vi "Measure.vi"() -> ()   [LabVIEW 2024]
uses:
  <vilib>/MakerHub/LINX/Public/Peripherals/Analog/Analog Read N Chans.vi
  <vilib>/MakerHub/LINX/Public/Peripherals/PWM/PWM Set Duty Cycle 1 Chan.vi
  <vilib>/MakerHub/LINX/Private/Local IO/LinxAnalogRead.vi
  <vilib>/MakerHub/LINX/Public/Utilities/Check Channel.vi
  <vilib>/MakerHub/LINX/Public/Utilities/Open Serial.vi
  Globals.vi
  <vilib>/MakerHub/LINX/Public/Peripherals/PWM/PWM Set Duty Cycle N Chans.vi
  <vilib>/addons/control/pid/pid.llb/PID (DBL).vi
  <vilib>/MakerHub/LINX/Private/Utilties/Generate Error.vi
  <vilib>/Utility/file.llb/Write Delimited Spreadsheet (string).vi
  <vilib>/MakerHub/LINX/LMH-LINX.lvlib
  <vilib>/addons/control/pid/NI_PID_pid.lvlib
  <vilib>/Analysis/NI_AALBase.lvlib
panel:
  out "Resistance":dbl(graph)
  out "TREF 2 Error":dbl
  out "TREF 2":dbl
  out "TREF 1 Error":dbl
  out "SC":dbl
  out "TREF 1":dbl
  in  "Target TC":dbl format="%.2f"
  in  "Target TH":dbl format="%.2f"
  out "Auto":bool
  in  "Start Auto":bool
  in  "TH End":dbl(knob)=100.0 step=10.0 scale=0.0..100.0
  in  "TH Start":dbl(knob)=40.0 step=10.0 scale=0.0..100.0
  out "VOUT - 1.25":dbl(knob) scale=-1.0..1.0
  out "TC":dbl(slide) scale=0.0..100.0
  out "TH":dbl(slide) scale=0.0..100.0
  out "Voltage":dbl(graph)
  out "TH":dbl(graph)
  in  "Save to File":bool
  out "VOUT - 1.25":dbl
  out "TC":dbl(graph)
  out "TC":dbl
  in  "Stop Button":bool
  out "TH":dbl
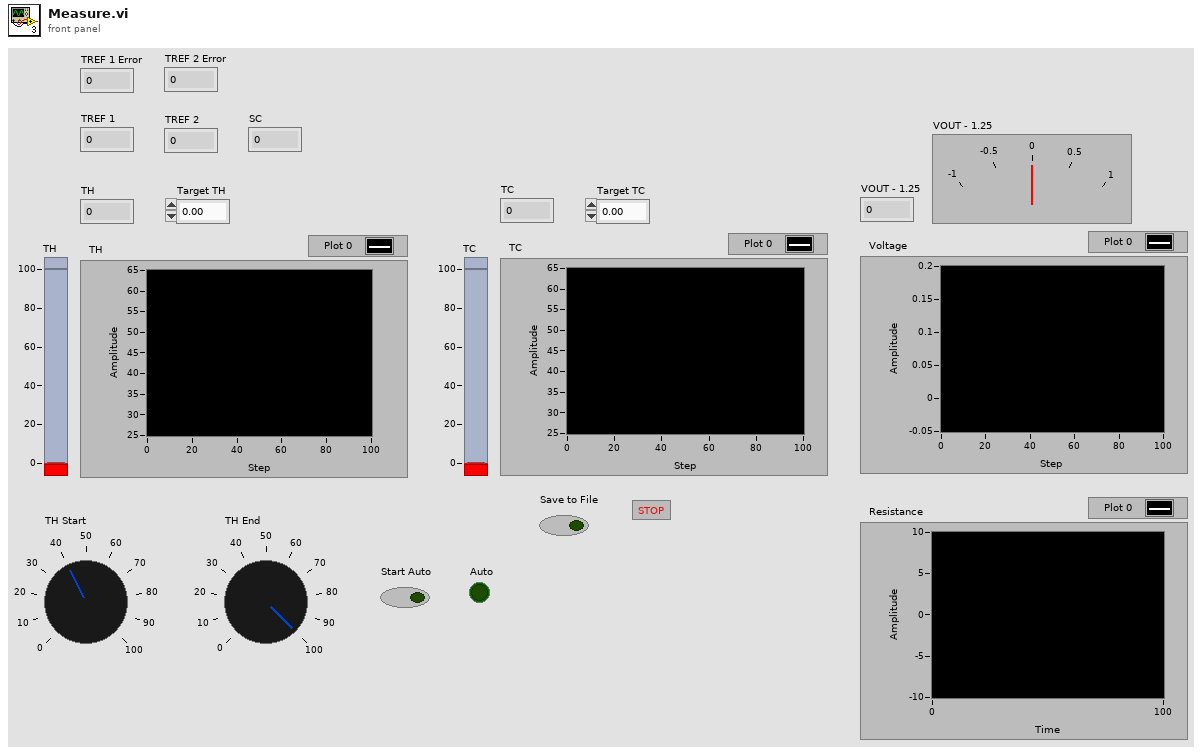
[diagram p1: front panel]
types:
  T1 = typedef "LMH-LINX.lvlib/LINX Ref.ctl" = cluster{"IO":T2, "Interface":T3, "LINX Device Config":T4}
  T2 = typedef "LMH-LINX.lvlib/Platform.ctl" = enum16{"Remote", "Local"}
  T3 = typedef "LMH-LINX.lvlib/Interface.ctl" = enum16{"Serial", "TCP"}
  T4 = typedef "LMH-LINX.lvlib/Device.lvlib/LINX Device Config.ctl" = cluster{"Interface":T3, "COM Port":refnum<visa-resource-name>, "TCP Configuration":T5, "Device Family":u8, "Device ID":u8, "Device Name":string, "TCP Ref":refnum<k5>, "Channels":T6}
  T5 = typedef "LMH-LINX.lvlib/Device.lvlib/TCP Config.ctl" = cluster{"IP Address":string, "Port":u16}
  T6 = typedef "LMH-LINX.lvlib/Channels.ctl" = cluster{"DI":u8[], "DO":u8[], "AI":u8[], "AO":u8[], "PWM":u8[], "QE":u8[], "UART":u8[], "I2C 2":u8[], "SPI":u8[], "CAN":u8[], "Servo":u8[], "AI Ref (V)":dbl, "AI Resolution (Bits)":u8, "AO Ref (V)":dbl, "AO Resolution (Bits)":u8}
  T7 = cluster{"proportional gain (Kc)":dbl, "integral time (Ti, min)":dbl, "derivative time (Td, min)":dbl}
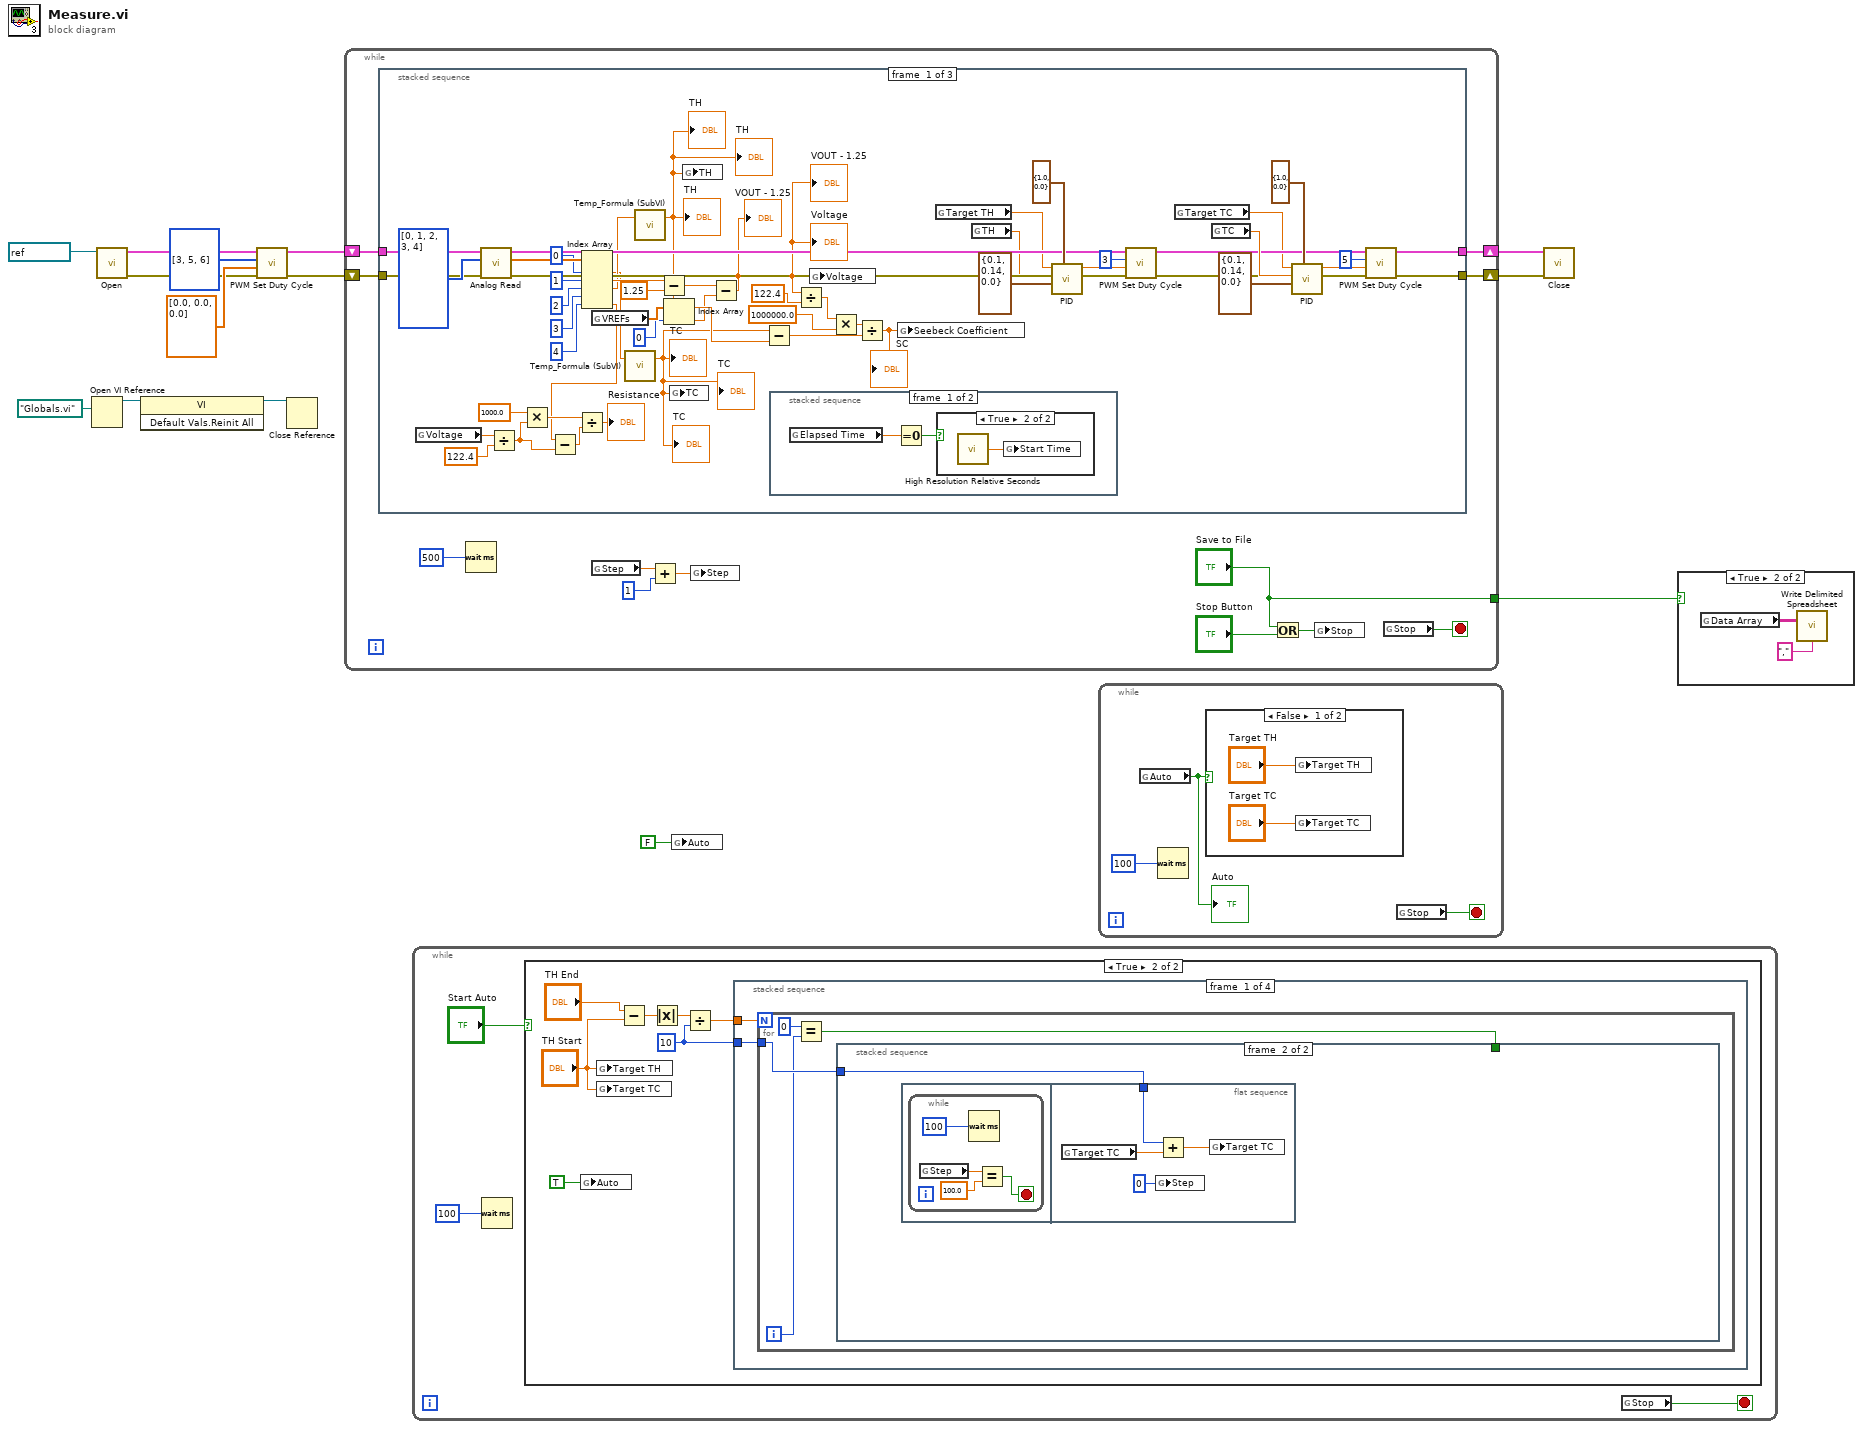
[diagram p0: block diagram]
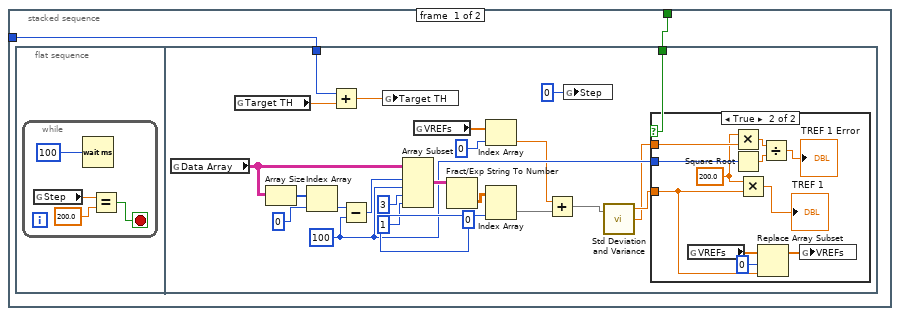
[diagram p3: hidden frame]
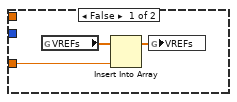
[diagram p4: hidden frame]
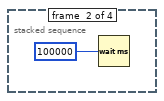
[diagram p5: hidden frame]
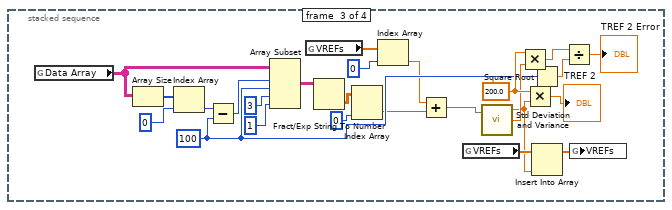
[diagram p6: hidden frame]
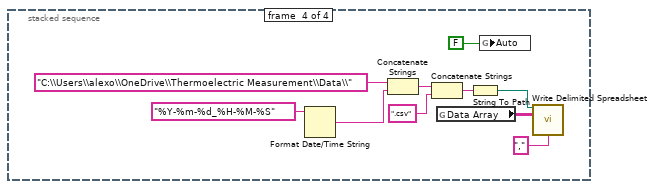
[diagram p7: hidden frame]
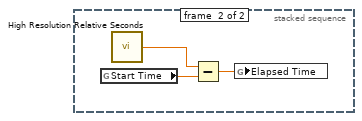
[diagram p11: hidden frame]
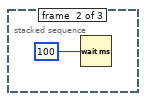
[diagram p12: hidden frame]
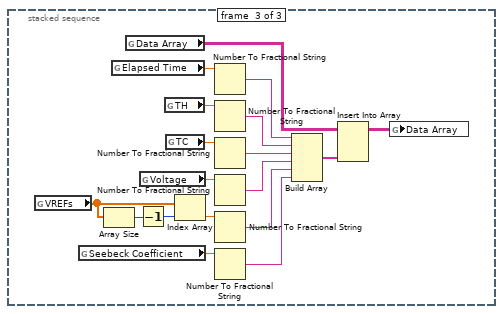
[diagram p13: hidden frame]
diagram:
  n1 = Open VI Reference(vi path=path "Globals.vi") -> (vi reference=w10:refnum<vi>)  [unwired: 5 in, 1 out]
  n2 = call-poly <vilib>:"Open.vi"("Serial Port"=refnum<visa-resource-name> "COM7") -> ("Error Out"=w2:errorcluster, "LINX Resource"=w5:T1)  [unwired: 8 in, 1 out]
  n3 = invoke class="VI" method="Default Vals.Reinit All"(reference=w10) -> (reference out=w9:refnum<vi>)  [unwired: 2 in, 2 out]
  n4 = call-poly <vilib>:"PWM Set Duty Cycle.vi"("Error In"=w2, "Duty Cycles"=dbl[] [0.0, 0.0, 0.0] ("Duty Cycle (0-1)"), "PWM Channels"=u8[] [3, 5, 6] ("PWM Channel"), "LINX Resource"=w5) -> ("Error Out"=w1:errorcluster, "LINX Resource"=w6:T1)  [unwired: 6 in]
  n5 = Close Reference(reference=w9) -> ()  [unwired: 1 in, 1 out]
  n6 = while {
    shift-right: [w25] -> w13
    shift-left: w6 -> [w26]
    shift-right: [w23] -> w12
    shift-left: w1 -> [w24]
    tunnel: ["Save to File"] -> w11
    stop <- w18 stop-if-true
    n7 = stacked-sequence {
      tunnel: w26 -> [w67 _ _]
      tunnel: [w56 _ _] -> w25
      tunnel: w24 -> [w66 _ _]
      tunnel: [w54 _ _] -> w23
      frame #0 {
        n8 = global read "Globals.vi" "Voltage"() -> (w34:dbl)
        n9 = call-poly <vilib>:"Analog Read.vi"("Error In"=w66, "AI Channel(s)"=i32[] [0, 1, 2, 3, 4], "LINX Resource"=w67) -> ("Error Out"=w64:errorcluster, "Voltages"=w75:dbl[], "LINX Resource"=w65:T1)  [unwired: 5 in, 1 out]
        n10 = Divide(x=w34, y=122.4) -> (x/y=w28:dbl)
        n11 = Multiply(x=1000.0 ("y"), y=w28) -> (x*y=w36:dbl)
        n12 = Index Array(array=w75, index #1=0 ("index"), index #2=1 ("index"), index #3=2 ("index"), index #4=3 ("index"), index #5=4 ("index")) -> (element #1=w41:dbl, element #2=w51:dbl, element #3=w42:dbl, element #5=w27:dbl)  [unwired: 1 out]
        n13 = Subtract(x=w27, y=w28) -> (x-y=w29:dbl)
        n14 = Divide(x=w36, y=w29) -> (x/y=→"Resistance":dbl)
        n15 = global read "Globals.vi" "VREFs"() -> (w40:dbl[])
        n16 = call "Temp_Formula (SubVI).vi"("In"=w41) -> ("Out"=w43:dbl)  [unwired: 1 in, 1 out]
        "TC" <- w43
        "TC" <- w43
        "TC" <- w43
        n17 = call "Temp_Formula (SubVI).vi"("In"=w42) -> ("Out"=w44:dbl)  [unwired: 1 in, 1 out]
        "TH" <- w44
        "TH" <- w44
        "TH" <- w44
        n18 = Subtract(x=w51, y=1.25) -> (x-y=w47:dbl)
        n19 = Index Array(array=w40, index=0) -> (element=w38:dbl)
        n20 = global write "Globals.vi" "TC"(w43) -> ()
        n21 = global write "Globals.vi" "TH"(w44) -> ()
        n22 = Subtract(x=w47, y=w38) -> (x-y=w37:dbl)
        "VOUT - 1.25" <- w37
        "Voltage" <- w37
        "VOUT - 1.25" <- w37
        n23 = Subtract(x=w43, y=w44) -> (x-y=w78:dbl)
        n24 = stacked-sequence {
          frame #0 {
            n25 = global read "Globals.vi" "Elapsed Time"() -> (w79:dbl)
            n26 = Equal To 0?(x=w79) -> (x = 0?=w80:bool)
            n27 = case shown="True" w80 {
              frame False {
              }
              frame True {
                n28 = call <vilib>:"High Resolution Relative Seconds.vi"() -> ("relative seconds"=w81:dbl)
                n29 = global write "Globals.vi" "Start Time"(w81) -> ()
              }
            }
          }
          frame #1 {
            n30 = global read "Globals.vi" "Start Time"() -> (w82:dbl)
            n31 = call <vilib>:"High Resolution Relative Seconds.vi"() -> ("relative seconds"=w83:dbl)
            n32 = Subtract(x=w83, y=w82) -> (x-y=w84:dbl)
            n33 = global write "Globals.vi" "Elapsed Time"(w84) -> ()
          }
        }
        n34 = Divide(x=w37, y=122.4) -> (x/y=w45:dbl)
        n35 = global write "Globals.vi" "Voltage"(w37) -> ()
        n36 = Multiply(x=w45, y=1000000.0) -> (x*y=w49:dbl)
        n37 = Divide(x=w49, y=w78) -> (x/y=w77:dbl)
        "SC" <- w77
        n38 = global write "Globals.vi" "Seebeck Coefficient"(w77) -> ()
        n39 = global read "Globals.vi" "Target TH"() -> (w53:dbl)
        n40 = global read "Globals.vi" "TH"() -> (w63:dbl)
        n41 = call-poly <vilib>:"PID.vi"("output range"=cluster{"output high":dbl, "output low":dbl} {"output high"=1.0, "output low"=0.0}, "PID gains"=T7 {"proportional gain (Kc)"=0.1, "integral time (Ti, min)"=0.14, "derivative time (Td, min)"=0.0}, "process variable"=w63, "setpoint"=w53) -> ("output"=w71:dbl)  [unwired: 6 in, 1 out]
        n42 = call-poly <vilib>:"PWM Set Duty Cycle.vi"("Error In"=w64, "Duty Cycle (0-1)"=w71, "PWM Channel"=u8 3, "LINX Resource"=w65) -> ("Error Out"=w55:errorcluster, "LINX Resource"=w57:T1)  [unwired: 6 in]
        n43 = global read "Globals.vi" "Target TC"() -> (w52:dbl)
        n44 = global read "Globals.vi" "TC"() -> (w58:dbl)
        n45 = call-poly <vilib>:"PID.vi"("output range"=cluster{"output high":dbl, "output low":dbl} {"output high"=1.0, "output low"=0.0}, "PID gains"=T7 {"proportional gain (Kc)"=0.1, "integral time (Ti, min)"=0.14, "derivative time (Td, min)"=0.0}, "process variable"=w58, "setpoint"=w52) -> ("output"=w62:dbl)  [unwired: 6 in, 1 out]
        n46 = call-poly <vilib>:"PWM Set Duty Cycle.vi"("Error In"=w55, "Duty Cycle (0-1)"=w62, "PWM Channel"=u8 5, "LINX Resource"=w57) -> ("Error Out"=w54:errorcluster, "LINX Resource"=w56:T1)  [unwired: 6 in]
      }
      frame #1 {
        n47 = Wait (ms)(milliseconds to wait=u32 100) -> ()  [unwired: 1 out]
      }
      frame #2 {
        n48 = global read "Globals.vi" "VREFs"() -> (w90:dbl[])
        n49 = global read "Globals.vi" "Seebeck Coefficient"() -> (w94:dbl)
        n50 = Array Size(array=w90) -> (size(s)=w89:i32)
        n51 = global read "Globals.vi" "Elapsed Time"() -> (w92:dbl)
        n52 = global read "Globals.vi" "Data Array"() -> (w102:string[][])
        n53 = Decrement(x=w89) -> (x-1=w88:i32)
        n54 = global read "Globals.vi" "Voltage"() -> (w99:dbl)
        n55 = global read "Globals.vi" "TH"() -> (w95:dbl)
        n56 = global read "Globals.vi" "TC"() -> (w97:dbl)
        n57 = Index Array(array=w90, index=w88) -> (element=w87:dbl)
        n58 = Number To Fractional String(number=w92) -> (F-format string=w93:string)  [unwired: 3 in]
        n59 = Number To Fractional String(number=w95) -> (F-format string=w96:string)  [unwired: 3 in]
        n60 = Number To Fractional String(number=w97) -> (F-format string=w98:string)  [unwired: 3 in]
        n61 = Number To Fractional String(number=w99) -> (F-format string=w100:string)  [unwired: 3 in]
        n62 = Number To Fractional String(number=w87) -> (F-format string=w86:string)  [unwired: 3 in]
        n63 = Number To Fractional String(number=w94) -> (F-format string=w91:string)  [unwired: 3 in]
        n64 = Build Array(w93, w96, w98, w100, w86, w91) -> (w101:string[])
        n65 = Insert Into Array(array=w102, new element=w101) -> (w103:string[][])  [unwired: 2 in]
        n66 = global write "Globals.vi" "Data Array"(w103) -> ()
      }
    }
    n67 = Wait (ms)(milliseconds to wait=u32 500) -> ()  [unwired: 1 out]
    n68 = global read "Globals.vi" "Step"() -> (w17:dbl)
    n69 = Add(x=w17, y=1) -> (x+y=w16:dbl)
    n70 = global write "Globals.vi" "Step"(w16) -> ()
    n71 = Or(x="Save to File", y="Stop Button") -> (x .or. y?=w19:bool)
    n72 = global write "Globals.vi" "Stop"(w19) -> ()
    n73 = global read "Globals.vi" "Stop"() -> (w18:bool)
  }
  n74 = while {
    stop <- w105 stop-if-true
    n75 = Wait (ms)(milliseconds to wait=u32 100) -> ()  [unwired: 1 out]
    n76 = case shown="True" "Start Auto" {
      frame False {
      }
      frame True {
        w108 = 10
        n77 = global write "Globals.vi" "Auto"(TRUE) -> ()
        n78 = global write "Globals.vi" "Target TH"("TH Start") -> ()
        n79 = global write "Globals.vi" "Target TC"("TH Start") -> ()
        n80 = Subtract(x="TH End", y="TH Start") -> (x-y=w111:dbl)
        n81 = Absolute Value(x=w111) -> (abs(x)=w110:dbl)
        n82 = Divide(x=w110, y=w108) -> (x/y=w107:dbl)
        n83 = stacked-sequence {
          tunnel: w107 -> [w115 _ _ _]
          tunnel: w108 -> [w114 _ _ _]
          frame #0 {
            n84 = for {
              N: w115 -> [_]
              tunnel: w114 -> [w119]
              i -> [w116]
              n85 = Equal?(x=0 ("y"), y=w116) -> (x = y?=w118:bool)
              n86 = stacked-sequence {
                tunnel: w119 -> [w121 w163]
                tunnel: w118 -> [w120 _]
                frame #0 {
                  n87 = flat-sequence {
                    tunnel: w121 -> [w146]
                    tunnel: w120 -> [w145]
                    frame #0 {
                      n88 = while {
                        stop <- w122 stop-if-true
                        n89 = global read "Globals.vi" "Step"() -> (w124:dbl)
                        n90 = Wait (ms)(milliseconds to wait=u32 100) -> ()  [unwired: 1 out]
                        n91 = Equal?(x=w124, y=200.0) -> (x = y?=w122:bool)
                      }
                    }
                    frame #1 {
                      w133 = 100 ("y")
                      n92 = global read "Globals.vi" "Data Array"() -> (w139:string[][])
                      n93 = global read "Globals.vi" "Target TH"() -> (w147:dbl)
                      n94 = Array Size(array=w139) -> (size(s)=w140:i32[])
                      n95 = Index Array(array=w140, index=0) -> (element=w141:i32)
                      n96 = Add(x=w146, y=w147) -> (x+y=w148:dbl)
                      n97 = Subtract(x=w141, y=w133) -> (x-y=w142:i32)
                      n98 = global write "Globals.vi" "Target TH"(w148) -> ()
                      n99 = Array Subset(array=w139, index (row)=w142, length (row)=w133, index (col)=3 ("index"), length (col)=1 ("length")) -> (w143:string[][])
                      n100 = global read "Globals.vi" "VREFs"() -> (w131:dbl[])
                      n101 = Fract/Exp String To Number(string=w143) -> (number=w144:dbl[][])  [unwired: 3 in, 1 out]
                      n102 = Index Array(array=w131, index=0) -> (element=w129:dbl)
                      n103 = Index Array(array=w144, index (col)=0 ("dimension size")) -> (element=w127:dbl[])  [unwired: 1 in]
                      n104 = Add(x=w129, y=w127) -> (x+y=w128:dbl[])
                      n105 = global write "Globals.vi" "Step"(0) -> ()
                      n106 = call <vilib>:"Std Deviation and Variance.vi"("X"=w128) -> ("mean"=w134:dbl, "standard deviation"=w132:dbl)  [unwired: 1 in, 1 out]
                      n107 = case shown="True" w145 {
                        tunnel: w134 -> [w149 w153]
                        tunnel: w133 -> [_ w160]
                        tunnel: w132 -> [_ w159]
                        frame False {
                          n108 = global read "Globals.vi" "VREFs"() -> (w150:dbl[])
                          n109 = Insert Into Array(array=w150, new element=w149) -> (w151:dbl[])  [unwired: 1 in]
                          n110 = global write "Globals.vi" "VREFs"(w151) -> ()
                        }
                        frame True {
                          w156 = 200.0 ("x")
                          n111 = global read "Globals.vi" "VREFs"() -> (w155:dbl[])
                          n112 = Multiply(x=w156, y=w159) -> (x*y=w161:dbl)
                          n113 = Square Root(x=w160) -> (sqrt(x)=w157:dbl)
                          n114 = Multiply(x=w156, y=w153) -> (x*y=→"TREF 1":dbl)
                          n115 = Replace Array Subset(array=w155, new element=w153, index=0) -> (w154:dbl[])
                          n116 = Divide(x=w161, y=w157) -> (x/y=→"TREF 1 Error":dbl)
                          n117 = global write "Globals.vi" "VREFs"(w154) -> ()
                        }
                      }
                    }
                  }
                }
                frame #1 {
                  n118 = flat-sequence {
                    tunnel: w163 -> [w169]
                    frame #0 {
                      n119 = while {
                        stop <- w164 stop-if-true
                        n120 = global read "Globals.vi" "Step"() -> (w166:dbl)
                        n121 = Wait (ms)(milliseconds to wait=u32 100) -> ()  [unwired: 1 out]
                        n122 = Equal?(x=w166, y=100.0) -> (x = y?=w164:bool)
                      }
                    }
                    frame #1 {
                      n123 = global read "Globals.vi" "Target TC"() -> (w170:dbl)
                      n124 = global write "Globals.vi" "Step"(0) -> ()
                      n125 = Add(x=w169, y=w170) -> (x+y=w171:dbl)
                      n126 = global write "Globals.vi" "Target TC"(w171) -> ()
                    }
                  }
                }
              }
            }
          }
          frame #1 {
            n127 = Wait (ms)(milliseconds to wait=u32 100000) -> ()  [unwired: 1 out]
          }
          frame #2 {
            w188 = 200.0 ("x")
            w183 = 100 ("y")
            n128 = global read "Globals.vi" "Data Array"() -> (w197:string[][])
            n129 = Array Size(array=w197) -> (size(s)=w195:i32[])
            n130 = Index Array(array=w195, index=0) -> (element=w193:i32)
            n131 = Subtract(x=w193, y=w183) -> (x-y=w192:i32)
            n132 = Array Subset(array=w197, index (row)=w192, length (row)=w183, index (col)=3 ("index"), length (col)=1 ("length")) -> (w189:string[][])
            n133 = global read "Globals.vi" "VREFs"() -> (w177:dbl[])
            n134 = Fract/Exp String To Number(string=w189) -> (number=w182:dbl[][])  [unwired: 3 in, 1 out]
            n135 = Index Array(array=w182, index (col)=0 ("dimension size")) -> (element=w173:dbl[])  [unwired: 1 in]
            n136 = Index Array(array=w177, index=0) -> (element=w175:dbl)
            n137 = Add(x=w175, y=w173) -> (x+y=w174:dbl[])
            n138 = global read "Globals.vi" "VREFs"() -> (w179:dbl[])
            n139 = call <vilib>:"Std Deviation and Variance.vi"("X"=w174) -> ("mean"=w178:dbl, "standard deviation"=w187:dbl)  [unwired: 1 in, 1 out]
            n140 = Multiply(x=w188, y=w187) -> (x*y=w186:dbl)
            n141 = Multiply(x=w188, y=w178) -> (x*y=→"TREF 2":dbl)
            n142 = Square Root(x=w183) -> (sqrt(x)=w185:dbl)
            n143 = Insert Into Array(array=w179, new element=w178) -> (w180:dbl[])  [unwired: 1 in]
            n144 = Divide(x=w186, y=w185) -> (x/y=→"TREF 2 Error":dbl)
            n145 = global write "Globals.vi" "VREFs"(w180) -> ()
          }
          frame #3 {
            n146 = Format Date/Time String(time format string (%c)="%Y-%m-%d_%H-%M-%S") -> (date/time string=w202:string)  [unwired: 2 in]
            n147 = Concatenate Strings("C:\\Users\\alexo\\OneDrive\\Thermoelectric Measurement\\Data\\" ("string"), w202) -> (w203:string)
            n148 = Concatenate Strings(w203, ".csv" ("string")) -> (w200:string)
            n149 = global read "Globals.vi" "Data Array"() -> (w206:string[][])
            n150 = String To Path(string=w200) -> (path=w199:path)
            n151 = global write "Globals.vi" "Auto"(FALSE) -> ()
            n152 = call-poly <vilib>:"Write Delimited Spreadsheet.vi"("file path (dialog if empty)"=w199, "2D data"=w206, "delimiter (\\t)"="," ("delimiter (\\t)")) -> ()  [unwired: 11 in, 2 out]
          }
        }
      }
    }
    n153 = global read "Globals.vi" "Stop"() -> (w105:bool)
  }
  n154 = global write "Globals.vi" "Auto"(FALSE) -> ()
  n155 = while {
    stop <- w209 stop-if-true
    n156 = global read "Globals.vi" "Auto"() -> (w210:bool)
    "Auto" <- w210
    n157 = Wait (ms)(milliseconds to wait=u32 100) -> ()  [unwired: 1 out]
    n158 = case shown="False" w210 {
      frame False {
        n159 = global write "Globals.vi" "Target TH"("Target TH") -> ()
        n160 = global write "Globals.vi" "Target TC"("Target TC") -> ()
      }
      frame True {
      }
    }
    n161 = global read "Globals.vi" "Stop"() -> (w209:bool)
  }
  n162 = call <vilib>:"Close.vi"("Error In"=w12, "LINX Resource"=w13) -> ()  [unwired: 9 in, 1 out]
  n163 = case shown="True" w11 {
    frame False {
    }
    frame True {
      n164 = global read "Globals.vi" "Data Array"() -> (w214:string[][])
      n165 = call-poly <vilib>:"Write Delimited Spreadsheet.vi"("2D data"=w214, "delimiter (\\t)"="," ("delimiter (\\t)")) -> ()  [unwired: 12 in, 2 out]
    }
  }
